vi "StateTransitionEdge_Create.vi"(0 "reference":refnum<class "StateTransitionEdge.lvclass">, 5 "error in (no error)":errorcluster) -> (14 "reference out":refnum<class "StateTransitionEdge.lvclass">, 19 "error out":errorcluster)   [LabVIEW 2020, in "StateTransitionEdge.lvclass"]
doc: "Creates and initializes a new StateTransitionEdge object.\n\nThis object should be destroyed using a StateTransitionEdge destructor VI or a virtual base class destructor VI.\n\n[GOOP 2.1]"
uses:
  <resource>/Framework/Providers/Open_GDS/UML/StateTransitionEdge_class/StateTransitionEdge.lvclass
  C:/Program Files (x86)/National Instruments/LabVIEW 2020/resource/Framework/Providers/Open_GDS/UML/ClassRelationshipEdge_class/ClassRelationshipEdge.lvclass
  C:/Program Files (x86)/National Instruments/LabVIEW 2020/resource/Framework/Providers/Open_GDS/UML/SegmentedLineEdge_class/SegmentedLineEdge.lvclass
  <resource>/Framework/Providers/Open_GDS/UML/ArrowHead_class/ArrowHeadType.ctl
  <resource>/Framework/Providers/Open_GDS/UML/BentStyle_class/BentStyleType.ctl
  <resource>/Framework/Providers/Open_GDS/UML/LineStyle_class/LineStyleType.ctl
  <resource>/Framework/Providers/Open_GDS/UML/ClassRelationshipEdge_class/ClassRelationshipEdge.lvclass
  <resource>/Framework/Providers/Open_GDS/UML/LineStyle_class/LineStyle.lvclass
  <resource>/Framework/Providers/Open_GDS/UML/ArrowHead_class/ArrowHead.lvclass
  <resource>/Framework/Providers/Open_GDS/UML/BentStyle_class/BentStyle.lvclass
  <resource>/Framework/Providers/Open_GDS/UML/SegmentedLineEdge_class/SegmentedLineEdge.lvclass
panel:
  # "The input reference should only\nbe wired when this method is called\nby a sub class constructor."
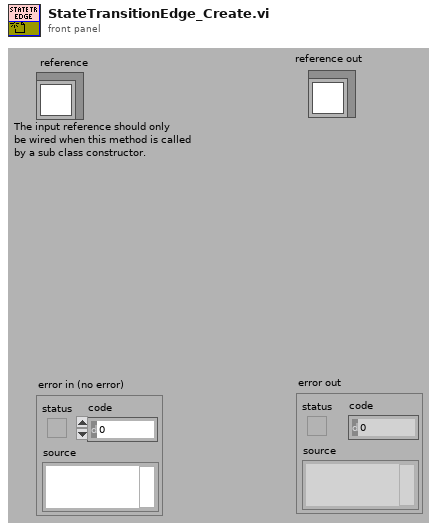
[diagram p1: front panel]
types:
  T1 = typedef "LineStyle.lvclass/LineStyleType.ctl" = enum16{"SOLID", "DOTTED"}
  T2 = typedef "BentStyle.lvclass/BentStyleType.ctl" = enum16{"STRAIGHT", "HV", "VH", "HVH", "VHV", "ARC"}
  T3 = typedef "ArrowHead.lvclass/ArrowHeadType.ctl" = enum16{"NONE", "TRIANGLE", "BLACK_TRIANGLE", "V", "HALF_V", "DIAMOND", "BLACK_DIAMOND"}
  T4 = typedef "ClassRelationshipEdge.lvclass/ObjectAttributes.ctl" = cluster{"bentStyleRef":refnum<class "BentStyle.lvclass">, "startConnectionOffset":cluster{"x":i32, "y":i32}, "endConnectionOffset":cluster{"x":i32, "y":i32}, "MidLineOffset":cluster{"x":i32, "y":i32}, "DepClass":T5}
  T5 = typedef "ReversedEngineering_ViDependencyDetailsType.ctl" = cluster{"ThisVIs/Ctls":path[], "Dependent_VIs/Ctls":path[]}
  T6 = typedef "SegmentedLineEdge.lvclass/ObjectAttributes.ctl" = cluster{"lineStyle":refnum<class "LineStyle.lvclass">, "startArrowHead":refnum<class "ArrowHead.lvclass">, "endArrowHead":refnum<class "ArrowHead.lvclass">, "startLabel":string, "midLabel":string, "endLabel":string, "MidLabelOffset":T7, "SplitWire":bool}
  T7 = typedef "Point Point2D.ctl" = cluster{"x":dbl, "y":dbl}
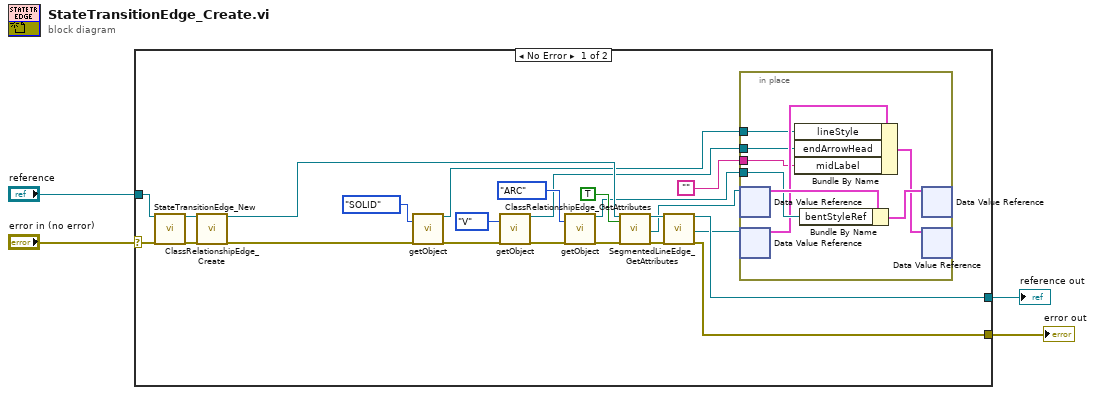
[diagram p0: block diagram]
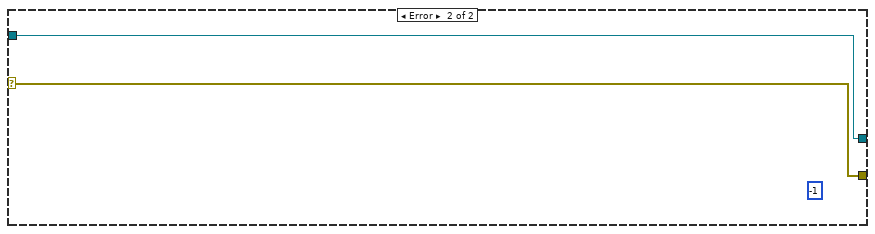
[diagram p2: hidden frame]
diagram:
  n1 = case shown="No Error" "error in (no error)" {
    selector: "error in (no error)" -> [w27 w37]
    tunnel: [w22 w36] -> w4
    tunnel: [w21 w37] -> w3
    tunnel: "reference" -> [w26 w36]
    frame No Error {
      n2 = call <resource>:"StateTransitionEdge_New.vi"("reference in"=w26, "error in (no error)"=w27) -> ("reference out"=w24:refnum<class "StateTransitionEdge.lvclass">, "error out"=w25:errorcluster)  [unwired: 2 in, 14 out]
      n3 = call <resource>:"ClassRelationshipEdge_Create.vi"("reference"=w24, "error in (no error)"=w25) -> ("reference out"=w23:refnum<class "StateTransitionEdge.lvclass">, "error out"=w20:errorcluster)  [unwired: 1 in, 15 out]
      n4 = call <resource>:"getObject.vi"("lineStyle"=LineStyleType."SOLID", "error in (no error)"=w20) -> ("reference out"=w7:refnum<class "LineStyle.lvclass">, "error out"=w18:errorcluster)  [unwired: 16 out]
      n5 = call <resource>:"getObject.vi"("arrowHead"=ArrowHeadType."V", "error in (no error)"=w18) -> ("reference out"=w6:refnum<class "ArrowHead.lvclass">, "error out"=w16:errorcluster)  [unwired: 16 out]
      n6 = call <resource>:"getObject.vi"("bentStyle"=BentStyleType."ARC", "error in (no error)"=w16) -> ("reference out"=w8:refnum<class "BentStyle.lvclass">, "error out"=w15:errorcluster)  [unwired: 16 out]
      n7 = call <resource>:"ClassRelationshipEdge_GetAttributes.vi"("reference in"=w23, "OnlyGetDvrReference(False)"=TRUE, "error in (no error)"=w15) -> ("reference out"=w12:refnum<class "StateTransitionEdge.lvclass">, "DataRef"=w10:refnum<data-value>, "error out"=w11:errorcluster)  [unwired: 13 in, 1 out]
      n8 = call <resource>:"SegmentedLineEdge_GetAttributes.vi"("reference in"=w12, "error in (no error)"=w11) -> ("reference out"=w22:refnum<class "StateTransitionEdge.lvclass">, "DataRef"=w9:refnum<data-value>, "error out"=w21:errorcluster)  [unwired: 14 in, 1 out]
      n9 = in-place {
        in-place-border: w8 -> [w34]
        in-place-border: w7 -> [w31]
        in-place-border: w6 -> [w30]
        in-place-border: "" -> [w29]
        n10 = in-place-dvr #1(w10) -> (w35:T4)  [unwired: 1 out]
        n11 = in-place-dvr #2(w9) -> (w32:T6)  [unwired: 1 out]
        n12 = Bundle By Name(cluster=w32, "lineStyle"=w31, "endArrowHead"=w30, "midLabel"=w29) -> (w28:T6)
        n13 = Bundle By Name(cluster=w35, "bentStyleRef"=w34) -> (w33:T4)
        n14 = in-place-dvr #1(w33) -> ()  [unwired: 2 out]
        n15 = in-place-dvr #2(w28) -> ()  [unwired: 2 out]
      }
    }
    frame Error {
      (unwired) -1 ("Nr of open handles")
    }
  }
  "error out" <- w3
  "reference out" <- w4
